vi "Initialize with Switch Parameters Core.vi"(8 "error in (no error)":errorcluster, 10 "Switch Parameters in":refnum<class "Abstract Switch Init Parameters.lvclass">, 11 "NI-SWITCH Consumer in":refnum<class "NI-SWITCH Consumer.lvclass">) -> (0 "error out":errorcluster, 3 "NI-SWITCH Consumer out":refnum<class "NI-SWITCH Consumer.lvclass">)   [LabVIEW 2020, in "NI-SWITCH Messaging.lvlib" / "NI-SWITCH Consumer.lvclass"]
uses:
  NI-SWITCH Consumer.lvclass
  Includes/CDMessaging.lvlibp/Switch/Abstract Switch Init Parameters/Abstract Switch Init Parameters.lvclass
  NI-SWITCH Init Parameters/NI-SWITCH Init Parameters.lvclass
  C:/Users/nitest/Desktop/Git 2020/niveristand-routing-and-faulting-message-library/Includes/CDMessaging.lvlibp/Switch/Abstract Switch Init Parameters/Abstract Switch Init Parameters.lvclass
  NI-SWITCH Consumer.lvclass/NI-SWITCH Consumer.ctl
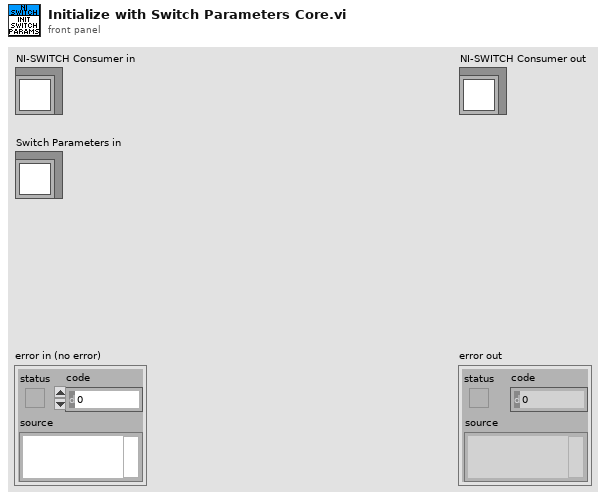
[diagram p1: front panel]
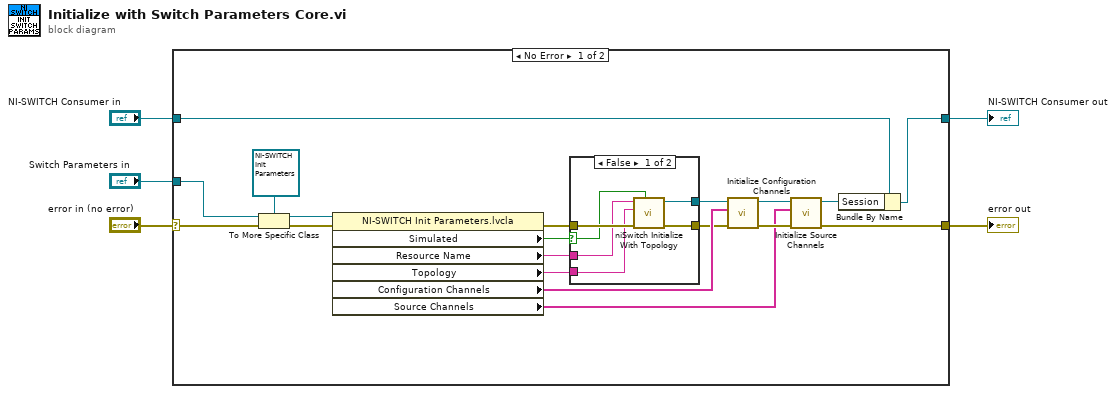
[diagram p0: block diagram]
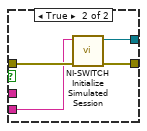
[diagram p2: hidden frame]
diagram:
  n1 = case shown="No Error" "error in (no error)" {
    selector: "error in (no error)" -> [w19 w36]
    tunnel: [w14 w36] -> w4
    tunnel: [w23 w35] -> w1
    tunnel: "NI-SWITCH Consumer in" -> [w24 w35]
    tunnel: "Switch Parameters in" -> [w21 _]
    frame No Error {
      n2 = To More Specific Class(target class=refnum<class "NI-SWITCH Init Parameters.lvclass"> refnum ("NI-SWITCH Messaging.lvlib:NI-SWITCH Init Parameters.lvclass"), reference=w21, error in=w19) -> (specific class reference=w20:refnum<class "NI-SWITCH Init Parameters.lvclass">, error out=w18:errorcluster)
      n3 = property class="NI-SWITCH Init Parameters.lvcla"(reference=w20, error in=w18) -> (error out=w22:errorcluster, "Simulated"=w8:bool, "Resource Name"=w7:string, "Topology"=w9:string, "Configuration Channels"=w13:string[], "Source Channels"=w12:string[])  [unwired: 1 out]
      n4 = case shown="False" w8 {
        selector: w8 -> [w26 _]
        tunnel: w22 -> [w30 w34]
        tunnel: [w29 w33] -> w11
        tunnel: [w28 w32] -> w10
        tunnel: w9 -> [w27 w31]
        tunnel: w7 -> [w25 _]
        frame False {
          n5 = call <instrlib>:"niSwitch Initialize With Topology.vi"("simulate (boolean value)"=w26, "error in (no error)"=w30, "topology name"=w27, "resource name"=w25) -> ("error out"=w29:errorcluster, "instrument handle out"=w28:refnum<k15>)  [unwired: 6 in]
        }
        frame True {
          n6 = call "NI-SWITCH Initialize Simulated Session.vi"("error in (no error)"=w34, "topology"=w31) -> ("error out"=w33:errorcluster, "NI-SWITCH session"=w32:refnum<k15>)  [unwired: 8 in]
        }
      }
      n7 = call "Initialize Configuration Channels.vi"("error in (no error)"=w11, "Configuration Channels"=w13, "Session in"=w10) -> ("error out"=w15:errorcluster, "Session out"=w17:refnum<k15>)  [unwired: 7 in]
      n8 = call "Initialize Source Channels.vi"("error in (no error)"=w15, "Source Channels"=w12, "Session in"=w17) -> ("error out"=w14:errorcluster, "Session out"=w16:refnum<k15>)  [unwired: 7 in]
      n9 = Bundle By Name(cluster=w24, "Session"=w16) -> (w23:refnum<class "NI-SWITCH Consumer.lvclass">)
    }
    frame Error {
    }
  }
  "error out" <- w4
  "NI-SWITCH Consumer out" <- w1
